vi "Get VIRef from Library.vi"(8 "error in (no error)":errorcluster, 10 "item name":string, 11 "library in":refnum<vi>) -> (0 "error out":errorcluster, 1 "found":bool, 2 "vi":refnum<vi>, 3 "library out":refnum<vi>)   [LabVIEW 2019, in "gRPC Template Creation Utility.lvlib"]
uses:
  gRPC Template Creation Utility.lvlib
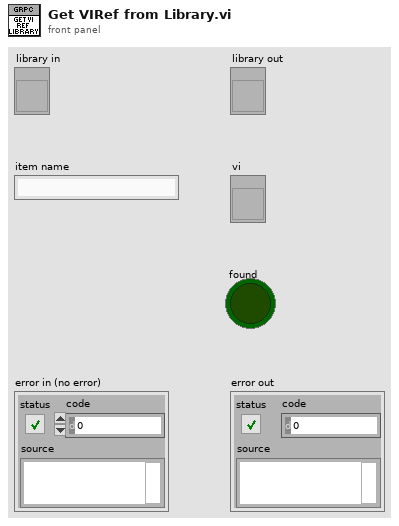
[diagram p1: front panel]
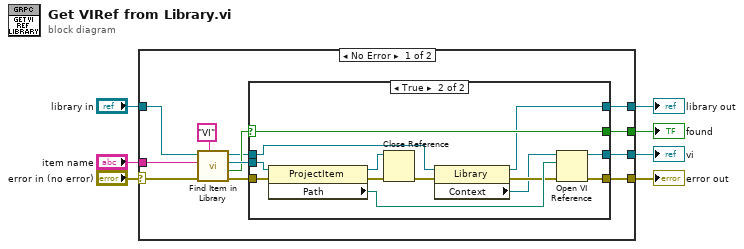
[diagram p0: block diagram]
diagram:
  n1 = case shown="No Error" "error in (no error)" {
    selector: "error in (no error)" -> [w13 w36]
    tunnel: "library in" -> [w17 w37]
    tunnel: "item name" -> [w15 _]
    tunnel: [w8 w37] -> w5
    tunnel: [w14 w36] -> w4
    tunnel: [w11 _] -> w2
    tunnel: [w10 _] -> w1
    frame No Error {
      n2 = call "Find Item in Library.vi"("Item Type"="VI", "error in (no error)"=w13, "Item Name"=w15, "Library item in"=w17) -> ("error out"=w19:errorcluster, "Found?"=w12:bool, "Project Item (Library Item)"=w18:refnum<vi>, "Library item out"=w9:refnum<vi>)  [unwired: 4 in]
      n3 = case shown="True" w12 {
        selector: w12 -> [w21 w32]
        tunnel: w19 -> [w22 w35]
        tunnel: w18 -> [_ w34]
        tunnel: [w22 w30] -> w14
        tunnel: [w21 w32] -> w11
        tunnel: [_ w31] -> w10
        tunnel: w9 -> [w20 w25]
        tunnel: [w20 w23] -> w8
        frame False {
        }
        frame True {
          n4 = property class="ProjectItem"(reference=w34, error in=w35) -> (reference out=w28:refnum<vi>, error out=w29:errorcluster, "Path"=w33:path)
          n5 = Close Reference(reference=w28, error in (no error)=w29) -> (error out=w27:errorcluster)
          n6 = property class="Library"(reference=w25, error in=w27) -> (reference out=w23:refnum<vi>, error out=w26:errorcluster, "Context"=w24:refnum<vi>)
          n7 = Open VI Reference(application reference (local)=w24, vi path=w33, error in (no error)=w26) -> (vi reference=w31:refnum<vi>, error out=w30:errorcluster)  [unwired: 3 in]
        }
      }
    }
    frame Error {
    }
  }
  "library out" <- w5
  "error out" <- w4
  "found" <- w2
  "vi" <- w1
